vi "GDSError_ReportError.vi"(5 "error in (no error)":errorcluster) -> (19 "error out":errorcluster)   [LabVIEW 2020]
doc: "You can use this VI to generate errors."
uses:
  <resource>/Framework/Providers/Open_GDS/ClassProviders/Common/Error/private/GDSError_LogCases.ctl
  <vilib>/Utility/error.llb/DialogType.ctl
  <resource>/Framework/Providers/Open_GDS/SubVIs/GOOP_ErrorCodes.ctl
panel:
  in  "Close":bool
  out "Error String":string
  # "A system error has occurred"
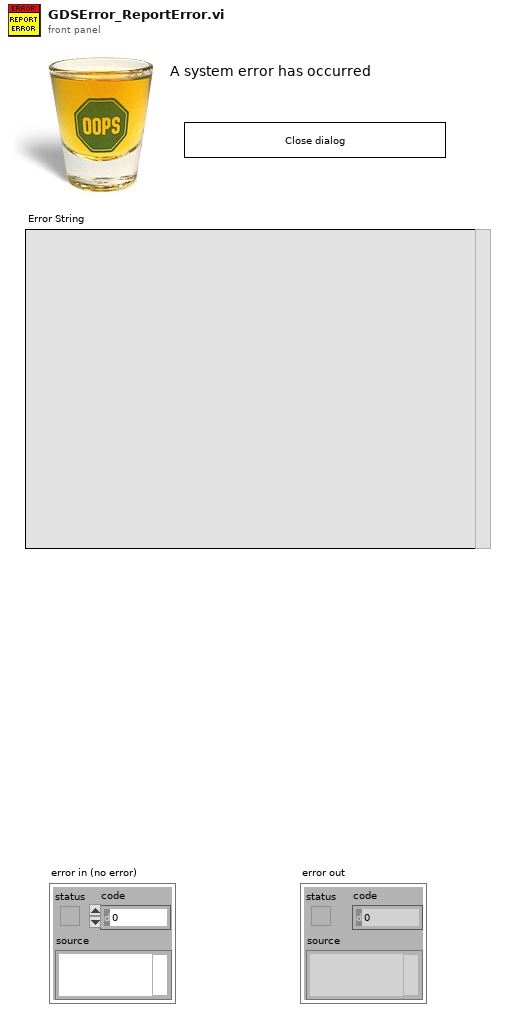
[diagram p1: front panel]
types:
  T1 = typedef "GDSError_LogCases.ctl" = enum16{"Init", "AddError", "ReadFirstError", "ReadLatestError", "ReadAllErrors", "ClearError", "ClearAllErrors"}
  T2 = enum32{"None", "Stop", "Question", "Exclamation", "Information"}
  T3 = cluster{"Counter":i32, "Text":string, "Email":string}
  T4 = enum16{"open", "replace", "create", "open or create", "replace or create", "replace or create with confirmation"}
  T5 = typedef "GOOP_ErrorCodes.ctl" = enum16{"LicenseFileMissing", "LicenseFileNotCorrect", "NoProductAccessGranted", "AgreementNoAccepted", "NoValidProviderFound", "LicenseExpired", "LanguageUndefined", "LanguageFileMissing", "LanguageFileChecksumError", "DublicateLanguageTranslation", "LanguageStringIDNotFound", "CommunityLimitReached", "ClassFileLocked", "ClassFileReadOnly", "ProjectNotValid"}
  T6 = typedef "DialogType.ctl" = u16
  T7 = typedef "LVRectTypeDef.ctl" = cluster{"Left":i16, "Top":i16, "Right":i16, "Bottom":i16}
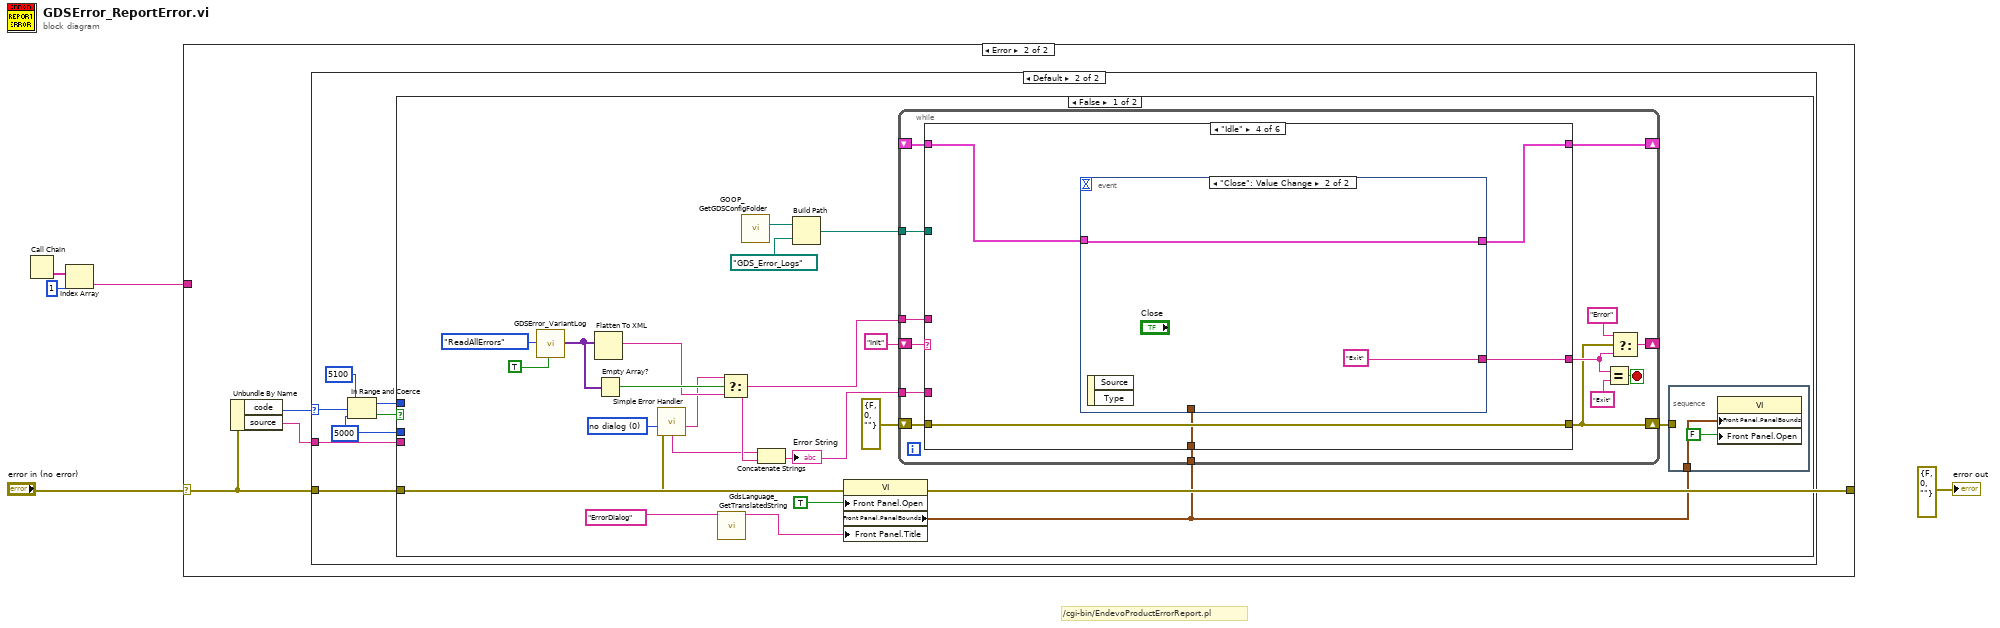
[diagram p0: block diagram]
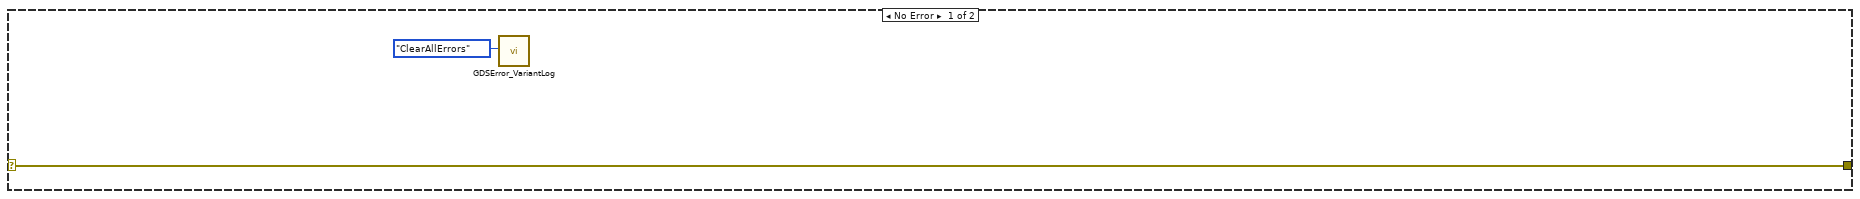
[diagram p2: hidden frame]
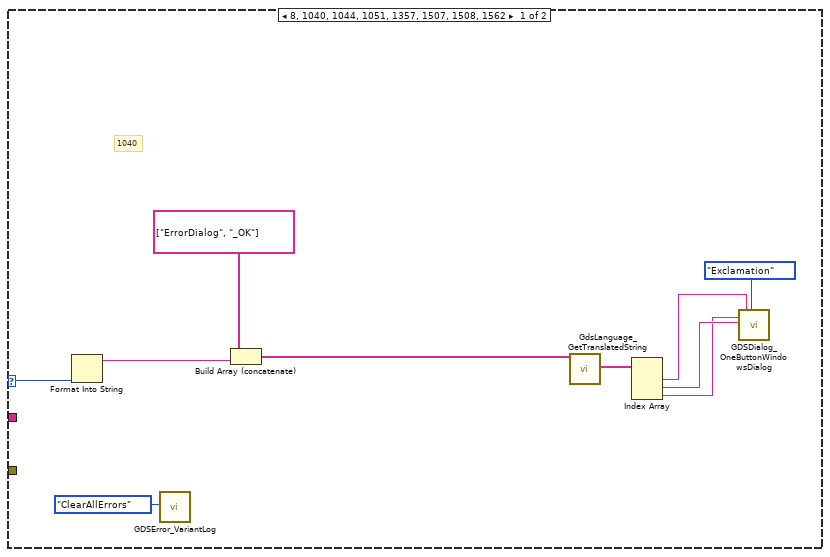
[diagram p3: hidden frame]
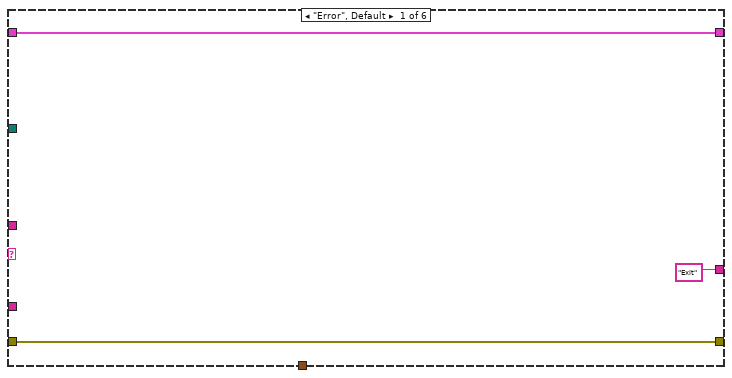
[diagram p4: hidden frame]
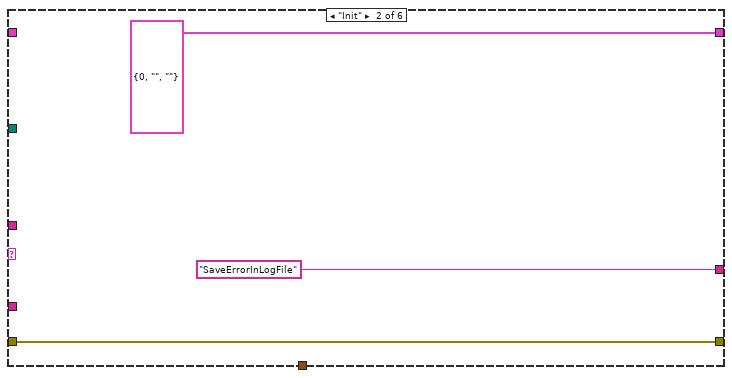
[diagram p5: hidden frame]
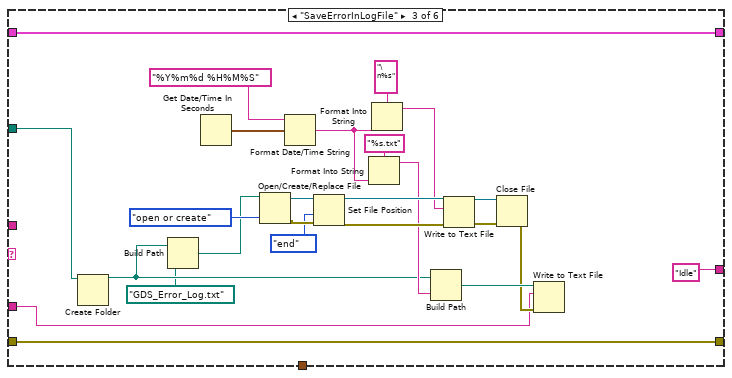
[diagram p6: hidden frame]
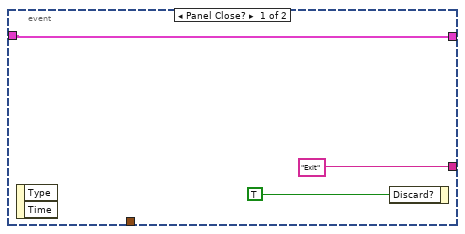
[diagram p7: hidden frame]
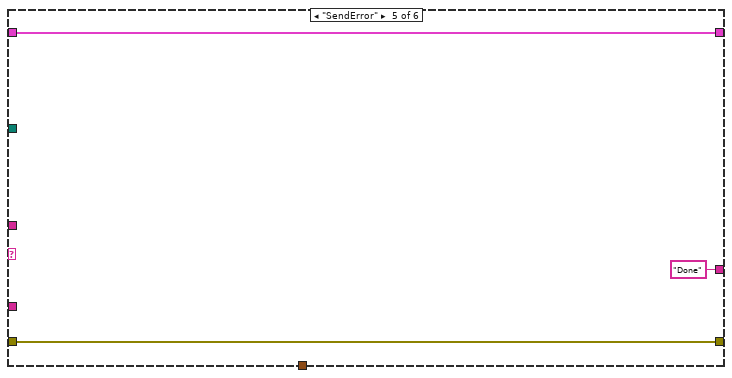
[diagram p8: hidden frame]
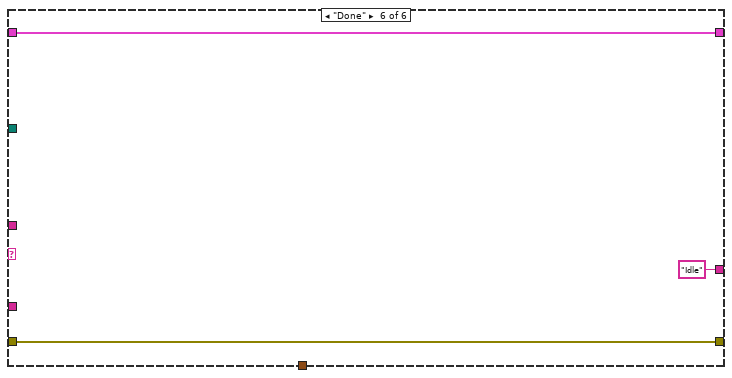
[diagram p9: hidden frame]
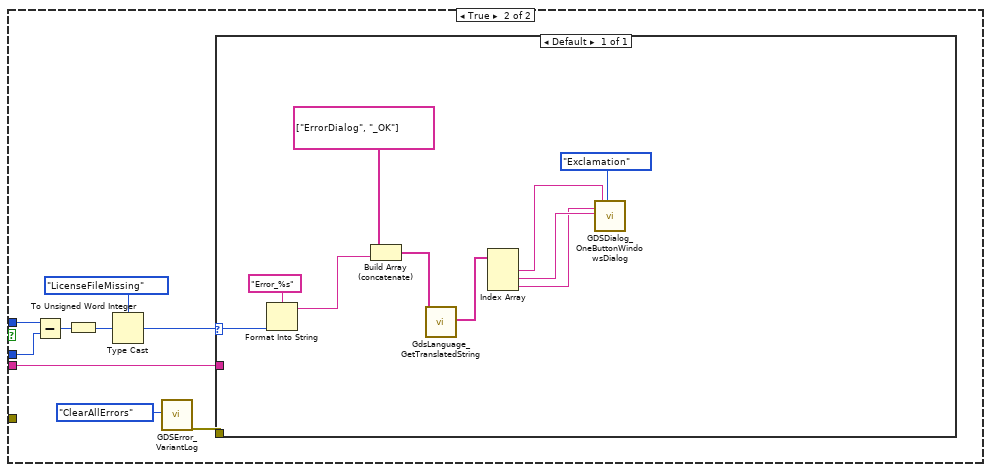
[diagram p10: hidden frame]
diagram:
  # "/cgi-bin/EndevoProductErrorReport.pl"
  n1 = Call Chain() -> (call chain=w4:string[])
  n2 = Index Array(array=w4, index=1) -> (element=w2:string)
  n3 = case shown="Error" "error in (no error)" {
    selector: "error in (no error)" -> [w7 w10]
    tunnel: [w7 w10] -> _
    tunnel: w2 -> [_ _]
    frame No Error {
      n4 = call <resource>:"GDSError_VariantLog.vi"("cases"=GDSError_LogCases."ClearAllErrors") -> ()  [unwired: 17 in, 2 out]
    }
    frame Error {
      n5 = Unbundle By Name(w10) -> ("code"=w9:i32, "source"=w8:string)
      n6 = case shown="Default" w9 {
        selector: w9 -> [w11 w22]
        tunnel: w10 -> [_ w27]
        tunnel: w8 -> [_ w21]
        frame 8, 1040, 1044, 1051, 1357, 1507, 1508, 1562 {
          # "1040"
          n7 = Format Into String(w11) -> (resulting string=w18:string)  [unwired: 3 in, 1 out]
          n8 = call <resource>:"GDSError_VariantLog.vi"("cases"=GDSError_LogCases."ClearAllErrors") -> ()  [unwired: 17 in, 2 out]
          n9 = Build Array (concatenate)(string[] ["ErrorDialog", "_OK"], w18) -> (w17:string[])
          n10 = call <resource>:"GdsLanguage_GetTranslatedString.vi"("StringID(s)"=w17) -> ("StringsOut"=w16:string[])  [unwired: 15 in, 3 out]
          n11 = Index Array(array=w16) -> (element #1=w15:string, element #2=w14:string, element #3=w13:string)  [unwired: 3 in]
          n12 = call <resource>:"GDSDialog_OneButtonWindowsDialog.vi"("UserText"=w13, "ButtonName"=w14, "DialogTitle"=w15, "Icon"=T2."Exclamation") -> ()  [unwired: 13 in, 3 out]
        }
        frame Default {
          w23 = 5000 ("y")
          n13 = In Range and Coerce(upper limit=5100, x=w22, lower limit=w23) -> (coerced(x)=w24:i32, In Range?=w25:bool)
          n14 = case shown="False" w25 {
            tunnel: w27 -> [w37 _]
            tunnel: w24 -> [_ w120]
            tunnel: w23 -> [_ w119]
            tunnel: w21 -> [_ w113]
            frame False {
              w45 = T6 0 items=["no dialog", "OK message", "continue or stop message", "OK message + warnings", "continue/stop + warnings"] ("type of dialog (OK msg:1)")
              n15 = call <resource>:"GDSError_VariantLog.vi"("cases"=GDSError_LogCases."ReadAllErrors", "DeleteWhenRead"=TRUE) -> ("ErrorArray"=w43:variant[])  [unwired: 16 in, 1 out]
              n16 = Flatten To XML(6:w43) -> (2:w42:string)
              n17 = Empty Array?(array=w43) -> (empty?=w44:bool)
              n18 = call <vilib>:"Simple Error Handler.vi"("type of dialog (OK msg:1)"=w45, "error in (no error)"=w37) -> ("source out"=w36:string, "message"=w34:string)  [unwired: 3 in, 3 out]
              n19 = call <resource>:"GdsLanguage_GetTranslatedString.vi"("StringID(s)"="ErrorDialog") -> ("FirstStringOut"=w32:string)  [unwired: 15 in, 3 out]
              n20 = Select(t=w36, s=w44, f=w42) -> (s? t:f=w35:string)
              n21 = call <resource>:"GOOP_GetGDSConfigFolder.vi"() -> ("GDSFolderPath"=w30:path)
              n22 = Concatenate Strings(w34, w35) -> (w31:string)
              "Error String" <- w31
              n23 = Build Path(base path=w30, name or relative path=path "GDS_Error_Logs" ("file path (use dialog)")) -> (appended path=w28:path)
              n24 = property class="VI"("Front Panel.Open"=TRUE ("Front Panel Window:Open"), "Front Panel.Title"=w32) -> ("Front Panel.PanelBounds"=w38:T7)  [unwired: 2 in, 2 out]
              n25 = while {
                shift-right: [w57] -> w39
                shift-left: errorcluster {"status"=FALSE, "code"=0, "source"=""} ("error IO") -> [w64]
                shift-right: [w62] -> _
                shift-left: "Init" -> [w63]
                shift-right: [w56] -> _
                shift-left: _ -> [w55]
                tunnel: w38 -> [w54]
                tunnel: w35 -> [w53]
                tunnel: w31 -> [w52]
                tunnel: w28 -> [w51]
                stop <- w61 stop-if-true
                n26 = case shown="\"Idle\"" w63 {
                  tunnel: w64 -> [w67 w69 w93 w99 w107 w109]
                  tunnel: [w67 w69 w93 w99 w107 w109] -> w57
                  tunnel: ["Exit" "SaveErrorInLogFile" "Idle" w100 "Done" "Idle"] -> w58
                  tunnel: [w65 T3 {"Counter"=0, "Text"="", "Email"=""} w95 w96 w106 w111] -> w56
                  tunnel: w55 -> [w65 _ w95 w97 w106 w111]
                  tunnel: w54 -> [_ _ _ w98 _ _]
                  tunnel: w53 -> [_ _ _ _ _ _]
                  tunnel: w52 -> [_ _ w72 _ _ _]
                  tunnel: w51 -> [_ _ w71 _ _ _]
                  frame "Error", Default {
                  }
                  frame "Init" {
                  }
                  frame "SaveErrorInLogFile" {
                    n27 = Create Folder(path (use dialog)=w71) -> (created path=w75:path)  [unwired: 2 in, 2 out]
                    n28 = Build Path(base path=w75, name or relative path=path "GDS_Error_Log.txt" ("file path (use dialog)")) -> (appended path=w73:path)
                    n29 = Get Date/Time In Seconds() -> (seconds since 1Jan1904=w87:timestamp)
                    n30 = Open/Create/Replace File(file path (use dialog)=w73, operation (0:open)=T4."open or create") -> (refnum out=w92:refnum<file>, error out=w91:errorcluster)  [unwired: 4 in, 1 out]
                    n31 = Format Date/Time String(time format string (%c)="%Y%m%d %H%M%S", seconds (now)=w87) -> (date/time string=w81:string)  [unwired: 1 in]
                    n32 = Set File Position(refnum=w92, from (0:start)=enum16{"start", "end", "current"}."end", error in=w91) -> (refnum out=w89:refnum<file>, error out=w88:errorcluster)  [unwired: 1 in]
                    n33 = Format Into String(format string="%s.txt", w81) -> (resulting string=w79:string)  [unwired: 2 in, 1 out]
                    n34 = Format Into String(format string="\n%s", w81) -> (resulting string=w84:string)  [unwired: 2 in, 1 out]
                    n35 = Build Path(base path=w75, name or relative path=w79) -> (appended path=w78:path)
                    n36 = Write to Text File(file (use dialog)=w89, text=w84, error in=w88) -> (refnum out=w82:refnum<file>, error out=w83:errorcluster)  [unwired: 1 in, 1 out]
                    n37 = Close File(refnum=w82, error in=w83) -> (error out=w77:errorcluster)  [unwired: 1 out]
                    n38 = Write to Text File(file (use dialog)=w78, text=w72, error in=w77) -> ()  [unwired: 1 in, 3 out]
                  }
                  frame "Idle" {
                    n39 = event shown="[1] \"Close\": Value Change" {
                      selector: _ -> [_ _]
                      dyn-events: _ -> [_ _]
                      timeout: _ -> [_ _]
                      tunnel: ["Exit" "Exit"] -> w100
                      tunnel: w98 -> [_ _]
                      tunnel: w97 -> [w101 w104]
                      tunnel: [w101 w104] -> w96
                      event Panel Close? {
                        n40 = event-data() -> ()  [unwired: 1 in, 2 out]
                        n41 = event-data("Discard?"=TRUE) -> ()  [unwired: 1 in, 1 out]
                      }
                      event "Close": Value Change {
                        n42 = event-data() -> ()  [unwired: 1 in, 2 out]
                      }
                    }
                  }
                  frame "SendError" {
                  }
                  frame "Done" {
                  }
                }
                n43 = Equal?(x=w58, y="Exit") -> (x = y?=w61:bool)
                n44 = Select(t="Error", s=w57, f=w58) -> (s? t:f=w62:string)
              }
              n45 = stacked-sequence {
                tunnel: w39 -> [_]
                tunnel: w38 -> [w50]
                frame #0 {
                  n46 = property class="VI"("Front Panel.PanelBounds"=w50, "Front Panel.Open"=FALSE ("Front Panel Window:Open")) -> ()  [unwired: 2 in, 2 out]
                }
              }
            }
            frame True {
              n47 = Subtract(x=w120, y=w119) -> (x-y=w118:i32)
              n48 = To Unsigned Word Integer(number=w118) -> (unsigned 16bit integer=w117:u16)
              n49 = Type Cast(type=GOOP_ErrorCodes."LicenseFileMissing" ("UserDefinedCodes(+5000)"), x=w117) -> (*(type *) &x=w115:T5)
              n50 = call <resource>:"GDSError_VariantLog.vi"("cases"=GDSError_LogCases."ClearAllErrors") -> ("error out"=w112:errorcluster)  [unwired: 17 in, 1 out]
              n51 = case shown="Default" w115 {
                selector: w115 -> [w121]
                tunnel: w113 -> [_]
                tunnel: w112 -> [_]
                frame Default {
                  n52 = Format Into String(format string="Error_%s", w121) -> (resulting string=w127:string)  [unwired: 2 in, 1 out]
                  n53 = Build Array (concatenate)(string[] ["ErrorDialog", "_OK"], w127) -> (w126:string[])
                  n54 = call <resource>:"GdsLanguage_GetTranslatedString.vi"("StringID(s)"=w126) -> ("StringsOut"=w125:string[])  [unwired: 15 in, 3 out]
                  n55 = Index Array(array=w125) -> (element #1=w124:string, element #2=w123:string, element #3=w122:string)  [unwired: 3 in]
                  n56 = call <resource>:"GDSDialog_OneButtonWindowsDialog.vi"("UserText"=w122, "ButtonName"=w123, "DialogTitle"=w124, "Icon"=T2."Exclamation") -> ()  [unwired: 13 in, 3 out]
                }
              }
            }
          }
        }
      }
    }
  }
  "error out" <- errorcluster {"status"=FALSE, "code"=0, "source"=""} ("error IO")
